vi "measure BT reference level.vi"(8 "error in (no error)":errorcluster, 11 "SA Measurement in":refnum<class "SA Measurement.lvclass">) -> (0 "error out":errorcluster, 3 "SA Measurement out":refnum<class "SA Measurement.lvclass">)   [LabVIEW 2023, in "Spectrum Analyzer.lvlib" / "SA Measurement.lvclass"]
uses:
  SA Measurement.lvclass
  SA Measurement.lvclass/SA Measurement.ctl
  TYPE DEFINITION/Keysight 9020A/TYPE Measurement Preset.ctl
  Spectrum Analyzer.lvlib
  Interface_Spectrum/Interface_Spectrum.lvclass
  TYPE DEFINITION/TYPE RBW and VBW Select.ctl
  TYPE DEFINITION/TYPE Marker Peak Search Type.ctl
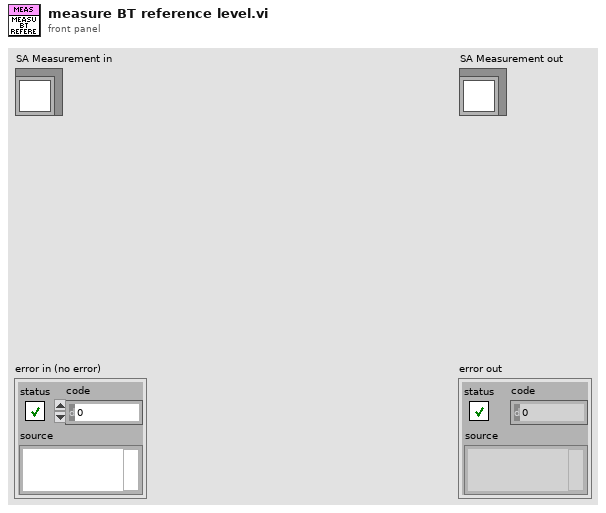
[diagram p1: front panel]
types:
  T1 = typedef "Spectrum Analyzer.lvlib/TYPE Marker Peak Search Type.ctl" = enum16{"Max", "Next Peak"}
  T2 = typedef "Spectrum Analyzer.lvlib/TYPE RBW and VBW Select.ctl" = enum16{"Res BW", "Video BW"}
  T3 = typedef "Spectrum Analyzer.lvlib/TYPE Measurement Preset.ctl" = enum16{"Sweep SA Mode", "Channel Power", "Occupied BW", "ACP", "Spurious Emission", "Spurious Emission Mask", "Burst Power (Transmit Power)"}
  T4 = typedef "Spectrum Analyzer.lvlib/TYPE Reference Level and Atten Param.ctl" = cluster{"Reference Level":dbl, "Atten":i32, "Atten Auto?":bool, "Reference Level Offset":dbl}
  T5 = typedef "Spectrum Analyzer.lvlib/TYPE Start and Stop Frequency.ctl" = cluster{"Start":dbl, "Stop":dbl}
  T6 = typedef "Spectrum Analyzer.lvlib/TYPE Display Trace Mode Select.ctl" = enum16{"Clear Write", "Max Hold", "Min Hold", "Average", "View"}
  T7 = typedef "Spectrum Analyzer.lvlib/TYPE Detect Mode Select.ctl" = enum16{"Det Auto (Normal)", "Auto Peak", "Positive Peak", "Negative Peak", "Sample", "RMS", "Average", "Quasipeak", "CISPR Average", "RMS Average"}
  T8 = cluster{"Trace Mode":T6, "Detector Type":T7, "Detect Auto?":bool}[]
  T9 = enum16{"Free Run", "Video (IF Envelop)", "RF Burst"}
  T10 = typedef "Spectrum Analyzer.lvlib/TYPE Marker Value.ctl" = cluster{"X-axis":dbl, "Y-axis":dbl}
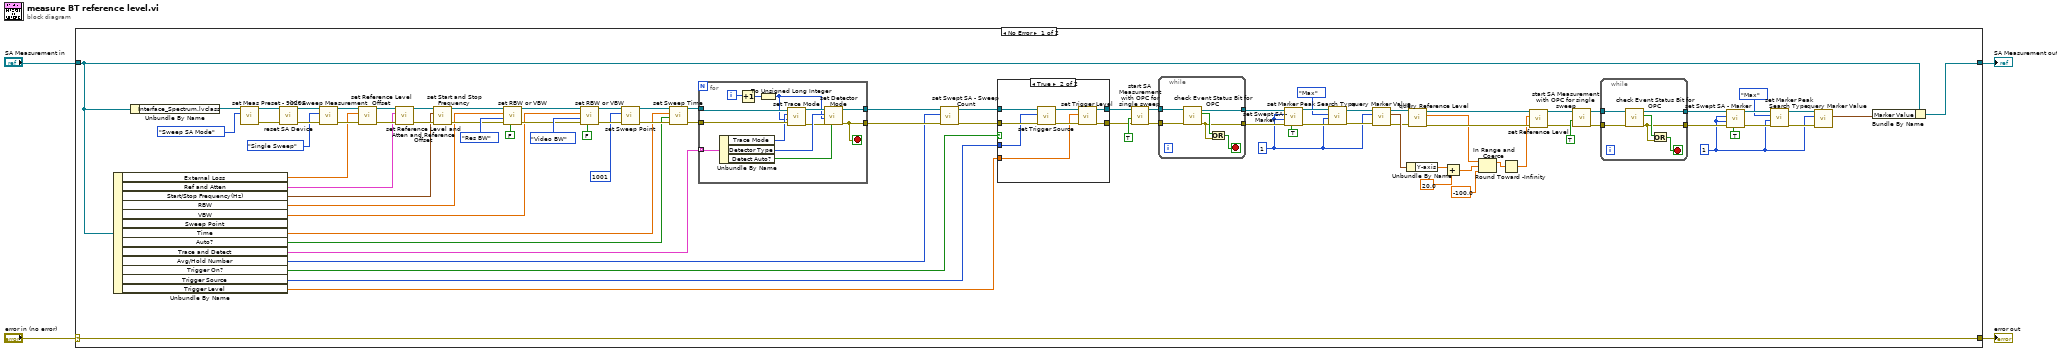
[diagram p0: block diagram]
diagram:
  n1 = case shown="No Error" "error in (no error)" {
    selector: "error in (no error)" -> [w92 w129]
    tunnel: [w92 w129] -> w3
    tunnel: [w33 w128] -> w1
    tunnel: "SA Measurement in" -> [w34 w128]
    frame No Error {
      w12 = 1 ("Index")
      w37 = 1 ("Index")
      n2 = Unbundle By Name(w34) -> ("External Loss"=w80:dbl, "Ref and Atten"=w79:T4, "Start/Stop Frequency(Hz)"=w76:T5, "RBW"=w67:dbl, "VBW"=w66:dbl, "Time"=w61:dbl, "Auto?"=w60:bool, "Trace and Detect"=w57:T8, "Avg/Hold Number"=w54:u32, "Trigger On?"=w53:bool, "Trigger Source"=w50:T9, "Trigger Level"=w49:dbl)  [unwired: 1 out]
      n3 = Unbundle By Name(w34) -> ("Interface_Spectrum.lvclass"=w91:refnum<class "Interface_Spectrum.lvclass">)
      n4 = call-dynamic "set Meas Preset - 9020A.vi"("Measurement Preset"=TYPE_Measurement_Preset."Sweep SA Mode", "Interface_Spectrum in"=w91) -> ("error out"=w88:errorcluster, "Interface_Spectrum out"=w89:refnum<class "Interface_Spectrum.lvclass">)  [unwired: 8 in]
      n5 = call-dynamic "reset SA Device.vi"("error in (no error)"=w88, "Interface_Spectrum in"=w89) -> ("error out"=w86:errorcluster, "Interface_Spectrum out"=w87:refnum<class "Interface_Spectrum.lvclass">)  [unwired: 8 in]
      n6 = call-dynamic "init Sweep Measurement.vi"("error in (no error)"=w86, "Sweep Measurement Mode"=enum16{"Single Sweep", "Continuous Sweep"}."Single Sweep", "Interface_Spectrum in"=w87) -> ("error out"=w83:errorcluster, "Interface_Spectrum out"=w84:refnum<class "Interface_Spectrum.lvclass">)  [unwired: 7 in]
      n7 = call-dynamic "set Reference Level Offset.vi"("error in (no error)"=w83, "Reference Level Offset"=w80, "Interface_Spectrum in"=w84) -> ("error out"=w81:errorcluster, "Interface_Spectrum out"=w82:refnum<class "Interface_Spectrum.lvclass">)  [unwired: 7 in]
      n8 = call-dynamic "set Reference Level and Atten and Reference Offset.vi"("error in (no error)"=w81, "Reference Level, Atten, Reference Offset"=w79, "Interface_Spectrum in"=w82) -> ("error out"=w77:errorcluster, "Interface_Spectrum out"=w78:refnum<class "Interface_Spectrum.lvclass">)  [unwired: 7 in]
      n9 = call-dynamic "set Start and Stop Frequency.vi"("error in (no error)"=w77, "Start/Stop Frequency(Hz)"=w76, "Interface_Spectrum in"=w78) -> ("error out"=w68:errorcluster, "Interface_Spectrum out"=w69:refnum<class "Interface_Spectrum.lvclass">)  [unwired: 7 in]
      n10 = call-dynamic "set RBW or VBW.vi"("BW Auto?"=FALSE, "error in (no error)"=w68, "BW Type"=TYPE_RBW_and_VBW_Select."Res BW", "BW Value (Hz)"=w67, "Interface_Spectrum in"=w69) -> ("error out"=w70:errorcluster, "Interface_Spectrum out"=w71:refnum<class "Interface_Spectrum.lvclass">)  [unwired: 5 in]
      n11 = call-dynamic "set RBW or VBW.vi"("BW Auto?"=FALSE, "error in (no error)"=w70, "BW Type"=TYPE_RBW_and_VBW_Select."Video BW", "BW Value (Hz)"=w66, "Interface_Spectrum in"=w71) -> ("error out"=w64:errorcluster, "Interface_Spectrum out"=w65:refnum<class "Interface_Spectrum.lvclass">)  [unwired: 5 in]
      n12 = call-dynamic "set Sweep Point.vi"("error in (no error)"=w64, "Sweep Point"=u32 1001, "Interface_Spectrum in"=w65) -> ("error out"=w62:errorcluster, "Interface_Spectrum out"=w63:refnum<class "Interface_Spectrum.lvclass">)  [unwired: 7 in]
      n13 = call-dynamic "set Sweep Time.vi"("error in (no error)"=w62, "Sweep Time Auto?"=w60, "Sweep Time(sec)"=w61, "Interface_Spectrum in"=w63) -> ("error out"=w58:errorcluster, "Interface_Spectrum out"=w59:refnum<class "Interface_Spectrum.lvclass">)  [unwired: 6 in]
      n14 = for {
        tunnel: w59 -> [w126]
        tunnel: w58 -> [w125]
        tunnel: w57 -> [w127] mode=indexing
        tunnel: [w115] -> w55
        tunnel: [w116] -> w56
        i -> [w124]
        stop <- w115 stop-if-true
        n15 = Unbundle By Name(w127) -> ("Trace Mode"=w122:T6, "Detector Type"=w120:T7, "Detect Auto?"=w117:bool)
        n16 = Increment(x=w124) -> (x+1=w123:i32)
        n17 = To Unsigned Long Integer(number=w123) -> (unsigned 32bit integer=w118:u32)
        n18 = call-dynamic "set Trace Mode.vi"("error in (no error)"=w125, "Trace Index"=w118, "Trace Mode"=w122, "Interface_Spectrum in"=w126) -> ("error out"=w119:errorcluster, "Interface_Spectrum out"=w121:refnum<class "Interface_Spectrum.lvclass">)  [unwired: 6 in]
        n19 = call-dynamic "set Detector Mode.vi"("Detect Auto?"=w117, "error in (no error)"=w119, "Trace Index"=w118, "Detector Type"=w120, "Interface_Spectrum in"=w121) -> ("error out"=w115:errorcluster, "Interface_Spectrum out"=w116:refnum<class "Interface_Spectrum.lvclass">)  [unwired: 5 in]
      }
      n20 = call-dynamic "set Swept SA - Sweep Count.vi"("error in (no error)"=w55, "Sweep Count"=w54, "Interface_Spectrum in"=w56) -> ("error out"=w51:errorcluster, "Interface_Spectrum out"=w52:refnum<class "Interface_Spectrum.lvclass">)  [unwired: 7 in]
      n21 = case shown="True" w53 {
        tunnel: w52 -> [w106 w114]
        tunnel: w51 -> [w105 w113]
        tunnel: w50 -> [_ w112]
        tunnel: w49 -> [_ w109]
        tunnel: [w106 w108] -> w36
        tunnel: [w105 w107] -> w35
        frame False {
        }
        frame True {
          n22 = call-dynamic "set Trigger Source.vi"("error in (no error)"=w113, "Trigger Source"=w112, "Interface_Spectrum in"=w114) -> ("error out"=w110:errorcluster, "Interface_Spectrum out"=w111:refnum<class "Interface_Spectrum.lvclass">)  [unwired: 7 in]
          n23 = call-dynamic "set Trigger Level.vi"("error in (no error)"=w110, "Trigger Level (dBm)"=w109, "Interface_Spectrum in"=w111) -> ("error out"=w107:errorcluster, "Interface_Spectrum out"=w108:refnum<class "Interface_Spectrum.lvclass">)  [unwired: 7 in]
        }
      }
      n24 = call-dynamic "start SA Measurement with OPC for single sweep.vi"("error in (no error)"=w35, "with OPC?"=TRUE, "Interface_Spectrum in"=w36) -> ("error out"=w46:errorcluster, "Interface_Spectrum out"=w47:refnum<class "Interface_Spectrum.lvclass">)  [unwired: 7 in]
      n25 = while {
        tunnel: w47 -> [w104]
        tunnel: w46 -> [w103]
        tunnel: [w100] -> w44
        tunnel: [w99] -> w45
        stop <- w101 stop-if-true
        n26 = call-dynamic "check Event Status Bit for OPC.vi"("error in (no error)"=w103, "Interface_Spectrum in"=w104) -> ("error out"=w100:errorcluster, "OPC Bit Changed?"=w102:bool, "Interface_Spectrum out"=w99:refnum<class "Interface_Spectrum.lvclass">)  [unwired: 7 in]
        n27 = Or(x=w102, y=w100) -> (x .or. y?=w101:bool)
      }
      n28 = call-dynamic "set Swept SA - Marker.vi"("On?"=TRUE, "error in (no error)"=w44, "trace"=w37, "Index"=w37, "Interface_Spectrum in"=w45) -> ("error out"=w41:errorcluster, "Interface_Spectrum out"=w42:refnum<class "Interface_Spectrum.lvclass">)  [unwired: 5 in]
      n29 = call-dynamic "set Marker Peak Search Type.vi"("error in (no error)"=w41, "Marker Index"=w37, "Peak Search Type"=TYPE_Marker_Peak_Search_Type."Max", "Interface_Spectrum in"=w42) -> ("error out"=w38:errorcluster, "Interface_Spectrum out"=w39:refnum<class "Interface_Spectrum.lvclass">)  [unwired: 6 in]
      n30 = call-dynamic "query Marker Value.vi"("error in (no error)"=w38, "Marker Index"=w37, "Interface_Spectrum in"=w39) -> ("error out"=w24:errorcluster, "Marker Value"=w25:T10, "Interface_Spectrum out"=w26:refnum<class "Interface_Spectrum.lvclass">)  [unwired: 6 in]
      n31 = Unbundle By Name(w25) -> ("Y-axis"=w31:dbl)
      n32 = call-dynamic "query Reference Level.vi"("error in (no error)"=w24, "Interface_Spectrum in"=w26) -> ("error out"=w28:errorcluster, "Ref Level"=w7:dbl, "Interface_Spectrum out"=w29:refnum<class "Interface_Spectrum.lvclass">)  [unwired: 7 in]
      n33 = Add(x=w31, y=20.0) -> (x+y=w6:dbl)
      n34 = In Range and Coerce(upper limit=w7, x=w6, lower limit=-100.0) -> (coerced(x)=w8:dbl)  [unwired: 1 out]
      n35 = Round Toward -Infinity(1:w8) -> (0:w27:dbl)
      n36 = call-dynamic "set Reference Level.vi"("error in (no error)"=w28, "Reference Level"=w27, "Interface_Spectrum in"=w29) -> ("error out"=w10:errorcluster, "Interface_Spectrum out"=w11:refnum<class "Interface_Spectrum.lvclass">)  [unwired: 7 in]
      n37 = call-dynamic "start SA Measurement with OPC for single sweep.vi"("error in (no error)"=w10, "with OPC?"=TRUE, "Interface_Spectrum in"=w11) -> ("error out"=w21:errorcluster, "Interface_Spectrum out"=w22:refnum<class "Interface_Spectrum.lvclass">)  [unwired: 7 in]
      n38 = while {
        tunnel: w22 -> [w98]
        tunnel: w21 -> [w97]
        tunnel: [w94] -> w19
        tunnel: [w93] -> w20
        stop <- w95 stop-if-true
        n39 = call-dynamic "check Event Status Bit for OPC.vi"("error in (no error)"=w97, "Interface_Spectrum in"=w98) -> ("error out"=w94:errorcluster, "OPC Bit Changed?"=w96:bool, "Interface_Spectrum out"=w93:refnum<class "Interface_Spectrum.lvclass">)  [unwired: 7 in]
        n40 = Or(x=w96, y=w94) -> (x .or. y?=w95:bool)
      }
      n41 = call-dynamic "set Swept SA - Marker.vi"("On?"=TRUE, "error in (no error)"=w19, "trace"=w12, "Index"=w12, "Interface_Spectrum in"=w20) -> ("error out"=w16:errorcluster, "Interface_Spectrum out"=w17:refnum<class "Interface_Spectrum.lvclass">)  [unwired: 5 in]
      n42 = call-dynamic "set Marker Peak Search Type.vi"("error in (no error)"=w16, "Marker Index"=w12, "Peak Search Type"=TYPE_Marker_Peak_Search_Type."Max", "Interface_Spectrum in"=w17) -> ("error out"=w13:errorcluster, "Interface_Spectrum out"=w14:refnum<class "Interface_Spectrum.lvclass">)  [unwired: 6 in]
      n43 = call-dynamic "query Marker Value.vi"("error in (no error)"=w13, "Marker Index"=w12, "Interface_Spectrum in"=w14) -> ("Marker Value"=w9:T10)  [unwired: 6 in, 2 out]
      n44 = Bundle By Name(cluster=w34, "Marker Value"=w9) -> (w33:refnum<class "SA Measurement.lvclass">)
    }
    frame Error {
    }
  }
  "error out" <- w3
  "SA Measurement out" <- w1
